vi "JSONRPC-BuildInfo.vi"(6 "keywords":string, 7 "authors":string, 8 "readables":T1(array[cluster]), 9 "writables":T1(array[cluster]), 10 "description":string, 11 "expId":string) -> (3 "info":string)   [LabVIEW 2015]
panel:
  # "BuildInfo"
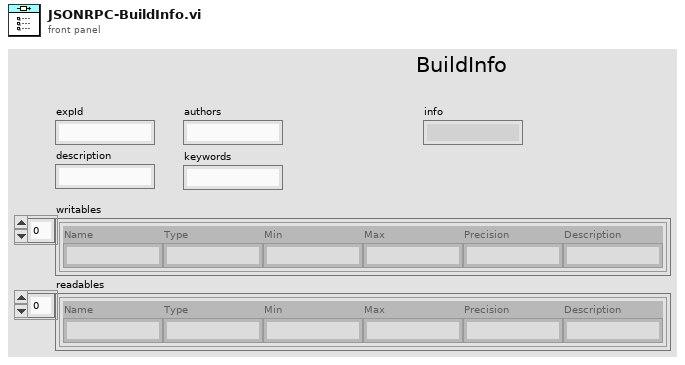
[diagram p1: front panel]
types:
  T1 = cluster{"Name":string, "Type":string, "Min":string, "Max":string, "Precision":string, "Description":string}[]
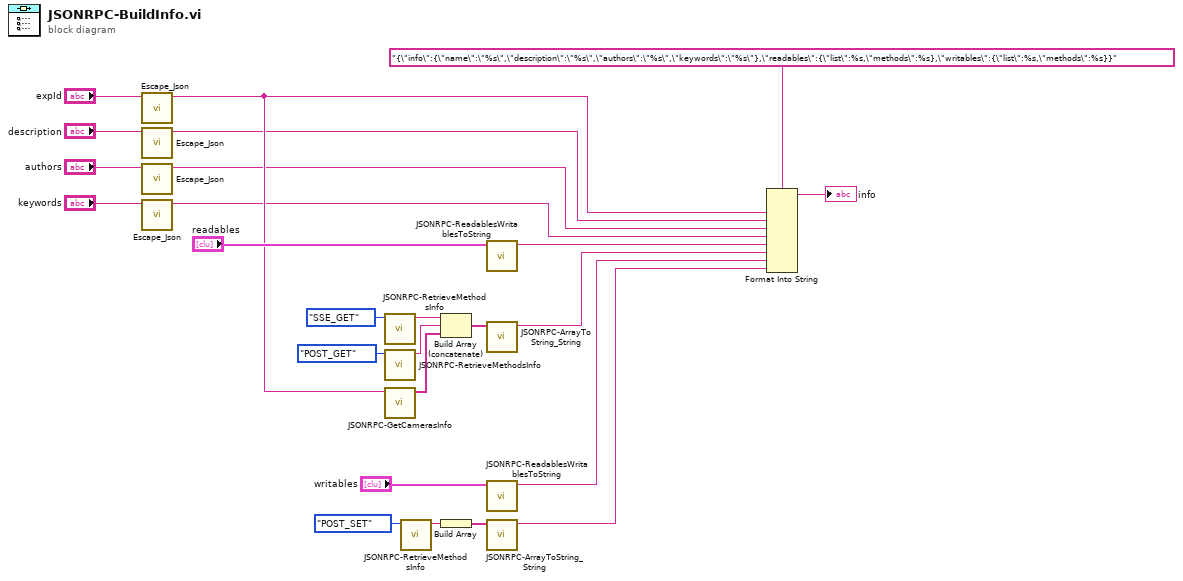
[diagram p0: block diagram]
diagram:
  n1 = call "Escape_Json.vi"("String"="expId") -> ("Json_string"=w4:string)  [unwired: 9 in]
  n2 = call "Escape_Json.vi"("String"="description") -> ("Json_string"=w3:string)  [unwired: 9 in]
  n3 = call "Escape_Json.vi"("String"="authors") -> ("Json_string"=w2:string)  [unwired: 9 in]
  n4 = call "Escape_Json.vi"("String"="keywords") -> ("Json_string"=w1:string)  [unwired: 9 in]
  n5 = call "JSONRPC-RetrieveMethodsInfo.vi"("Method"=enum16{"POST_SET", "POST_GET", "SSE_GET"}."SSE_GET") -> ("Output"=w18:string)  [unwired: 10 in]
  n6 = call "JSONRPC-RetrieveMethodsInfo.vi"("Method"=enum16{"POST_SET", "POST_GET", "SSE_GET"}."POST_GET") -> ("Output"=w19:string)  [unwired: 10 in]
  n7 = call "JSONRPC-GetCamerasInfo.vi"("expId"=w4) -> ("Output"=w9:string[])  [unwired: 10 in]
  n8 = call "JSONRPC-RetrieveMethodsInfo.vi"("Method"=enum16{"POST_SET", "POST_GET", "SSE_GET"}."POST_SET") -> ("Output"=w20:string)  [unwired: 10 in]
  n9 = Build Array (concatenate)(w18, w19, w9) -> (w14:string[])
  n10 = Build Array(w20) -> (w21:string[])
  n11 = call "JSONRPC-ReadablesWritablesToString.vi"("readables/writables"="readables") -> ("Output"=w10:string)  [unwired: 10 in]
  n12 = call "JSONRPC-ArrayToString_String.vi"("Array"=w14) -> ("Output"=w11:string)  [unwired: 10 in]
  n13 = call "JSONRPC-ReadablesWritablesToString.vi"("readables/writables"="writables") -> ("Output"=w12:string)  [unwired: 10 in]
  n14 = call "JSONRPC-ArrayToString_String.vi"("Array"=w21) -> ("Output"=w13:string)  [unwired: 10 in]
  n15 = Format Into String(format string="{\"info\":{\"name\":\"%s\",\"description\":\"%s\",\"authors\":\"%s\",\"keywords\":\"%s\"},\"readables\":{\"list\":%s,\"methods\":%s},\"writables\":{\"list\":%s,\"methods\":%s}}", w4, w3, w2, w1, w10, w11, w12, w13) -> (resulting string=→"info":string)  [unwired: 2 in, 1 out]
